vi "CheckAuth.vi"(8 "error in (no error)":errorcluster, 10 "ITool in":refnum<class "ITool.lvclass">, 11 "LabVIEW Web Service Request":refnum<class "Web Request.lvclass"> caption="LabVIEW Web Service Request in") -> (0 "error out":errorcluster, 1 "isAuthrized":bool, 2 "ITool out":refnum<class "ITool.lvclass">, 3 "LabVIEW Web Service Request out":refnum<class "Web Request.lvclass">)   [LabVIEW 2017]
uses:
  <vilib>/wsapi/Web Request.lvclass
  ITool/ITool.lvclass
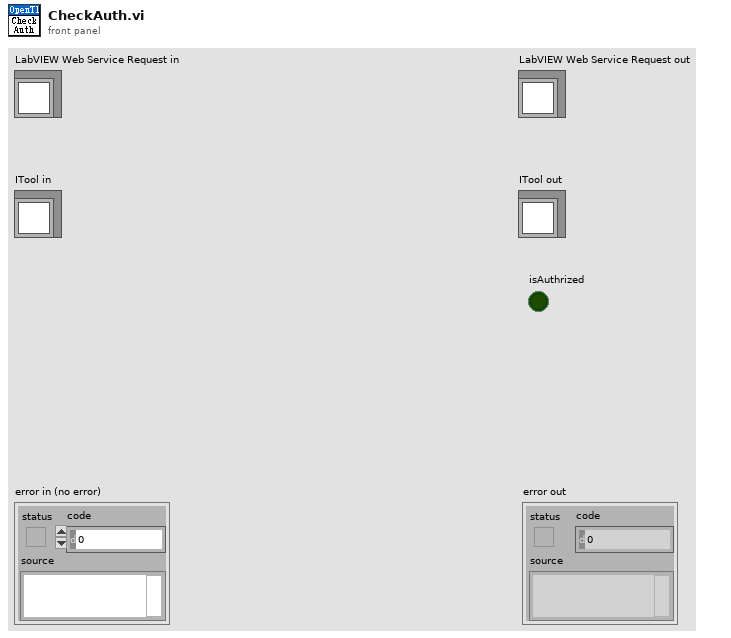
[diagram p1: front panel]
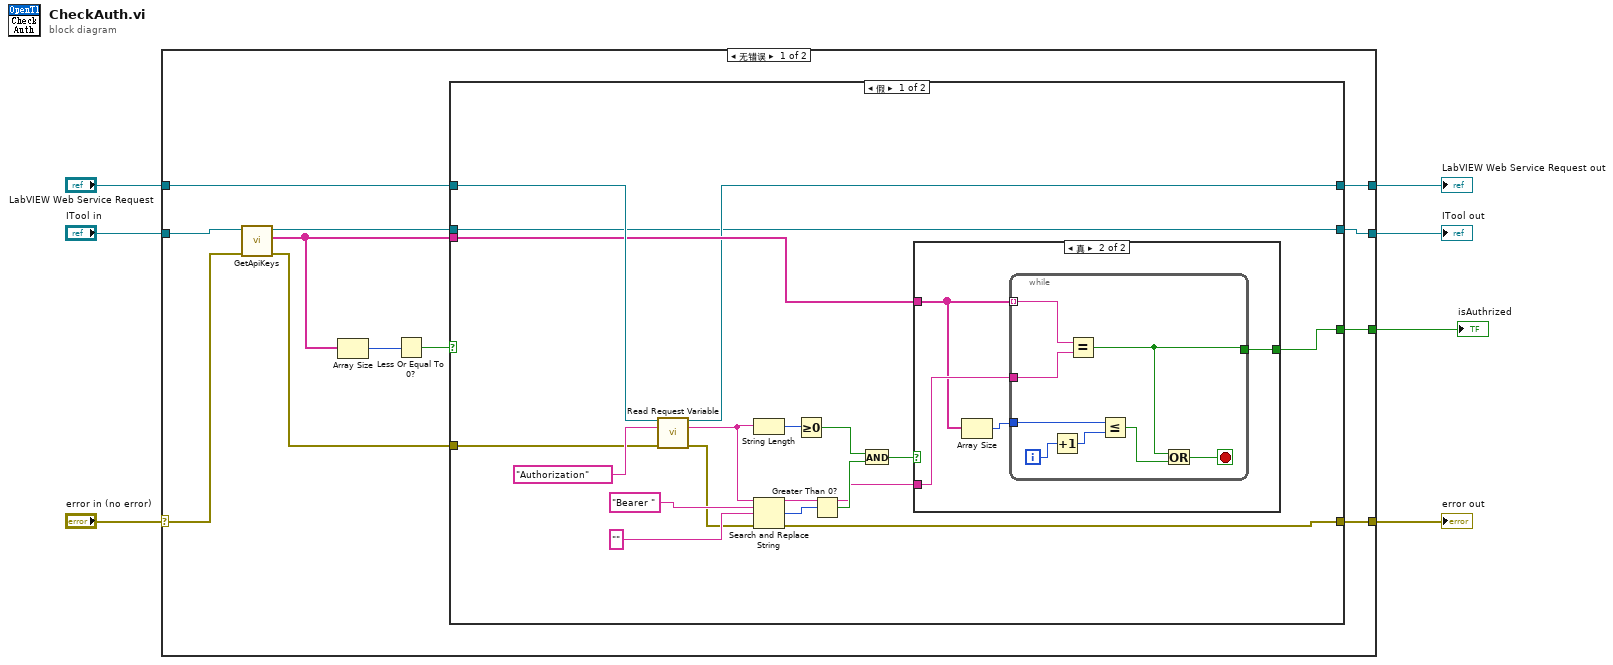
[diagram p0: block diagram]
diagram:
  n1 = case shown="无错误" "error in (no error)" {
    selector: "error in (no error)" -> [w18 w57]
    tunnel: [w11 w57] -> w6
    tunnel: "ITool in" -> [w19 w55]
    tunnel: [w17 _] -> w5
    tunnel: "LabVIEW Web Service Request" -> [w16 w56]
    tunnel: [w10 w56] -> w2
    tunnel: [w8 w55] -> w1
    frame No Error {
      n2 = call "GetApiKeys.vi"("error in (no error)"=w18, "ITool in"=w19) -> ("error out"=w12:errorcluster, "ApiKeys"=w15:string[], "ITool out"=w9:refnum<class "ITool.lvclass">)  [unwired: 7 in]
      n3 = Array Size(array=w15) -> (size(s)=w14:i32)
      n4 = Less Or Equal To 0?(x=w14) -> (x <= 0?=w13:bool)
      n5 = case shown="假" w13 {
        selector: w13 -> [_ w54]
        tunnel: [w32 w54] -> w17
        tunnel: w16 -> [w36 w52]
        tunnel: w15 -> [w33 _]
        tunnel: w12 -> [w34 w53]
        tunnel: [w22 w53] -> w11
        tunnel: [w21 w52] -> w10
        tunnel: w9 -> [w20 w51]
        tunnel: [w20 w51] -> w8
        frame False {
          n6 = call <vilib>:"Read Request Variable.vi"("LabVIEW Web Service Request"=w36, "variable name"="Authorization", "error in (no error)"=w34) -> ("LabVIEW Web Service Request out"=w21:refnum<class "Web Request.lvclass">, "value"=w28:string, "error out"=w27:errorcluster)  [unwired: 10 in]
          n7 = String Length(string=w28) -> (length=w35:i32)
          n8 = Search and Replace String(input string=w28, search string="Bearer " ("搜索字符串"), replace string="" ("替换字符串(\"\")"), error in=w27) -> (result string=w23:string, number of replacements=w29:i32, error out=w22:errorcluster)  [unwired: 4 in, 1 out]
          n9 = Greater Or Equal To 0?(x=w35) -> (x >= 0?=w26:bool)
          n10 = Greater Than 0?(x=w29) -> (x > 0?=w25:bool)
          n11 = And(x=w26, y=w25) -> (x .and. y?=w24:bool)
          n12 = case shown="真" w24 {
            selector: w24 -> [w38 _]
            tunnel: [w38 w42] -> w32
            tunnel: w33 -> [_ w40]
            tunnel: w23 -> [_ w41]
            frame False {
            }
            frame True {
              n13 = Array Size(array=w40) -> (size(s)=w39:i32)
              n14 = while {
                tunnel: w40 -> [w50] mode=indexing
                tunnel: w41 -> [w49]
                tunnel: [w43] -> w42
                tunnel: w39 -> [w48]
                i -> [w47]
                stop <- w44 stop-if-true
                n15 = Increment(x=w47) -> (x+1=w46:i32)
                n16 = Equal?(x=w50, y=w49) -> (x = y?=w43:bool)
                n17 = Less Or Equal?(x=w48, y=w46) -> (x <= y?=w45:bool)
                n18 = Or(x=w43, y=w45) -> (x .or. y?=w44:bool)
              }
            }
          }
        }
        frame True {
        }
      }
    }
    frame Error {
    }
  }
  "error out" <- w6
  "isAuthrized" <- w5
  "LabVIEW Web Service Request out" <- w2
  "ITool out" <- w1
